vi "Import FPGA Addon Configuration.vi"(8 "error in":errorcluster, 10 "configuration file path":path, 11 "FPGA addon refnum in":T1=18446744073709551615 format="%.0x") -> (0 "error out":errorcluster, 3 "FPGA addon refnum out":T1=18446744073709551615 format="%.0x")   [LabVIEW 2020, in "Scripting API.lvlib"]
doc: "Imports and applies the FPGA addon configuration to the target custom device. The wired path must lead to a valid \".dat\" file, otherwise this VI will return an error."
uses:
  Scripting API.lvlib
  <vilib>/NI VeriStand/Custom Device API/Custom Device Item Ref.ctl
  Addon/Addon Shared/Types/FG Action.ctl
  Addon/Addon Shared/Types/FPGA Settings.ctl
  Addon/Addon Shared/SubVIs/Constants.vi
  <vilib>/NI VeriStand/Custom Device API/NI VeriStand - Get Item Property.vi
  <vilib>/NI VeriStand/Custom Device API/Get Item Property (Path).vi
  <vilib>/NI VeriStand/Custom Device API/Get Item Property (String).vi
  <vilib>/NI VeriStand/Custom Device API/Get Item Property (Boolean).vi
  <vilib>/NI VeriStand/Custom Device API/NI VeriStand - Set Item Property.vi
  <vilib>/NI VeriStand/Custom Device API/Set Item Property (Path).vi
  <vilib>/NI VeriStand/Custom Device API/Set Item Property (String).vi
  <vilib>/NI VeriStand/Custom Device API/Set Item Property (Boolean).vi
  <vilib>/NI/NI VeriStand Custom Device Import and Export Tool/ImportExport.lvlib
  Addon/Addon Shared/FPGA Addon Shared.lvlib
  <vilib>/NI VeriStand/Custom Device API/Custom Device API.lvlib
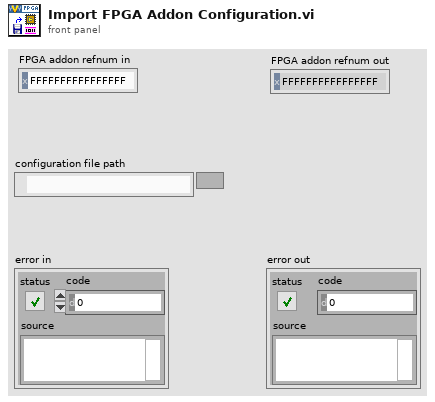
[diagram p1: front panel]
types:
  T1 = typedef "Custom Device API.lvlib/Custom Device Item Ref.ctl" = u64
  T2 = typedef "FPGA Addon Shared.lvlib/FPGA Settings.ctl" = cluster{"Bitfile path":path, "RIO Device Address":string, "Group":bool}
  T3 = typedef "FPGA Addon Shared.lvlib/FG Action.ctl" = enum8{"GET", "SET"}
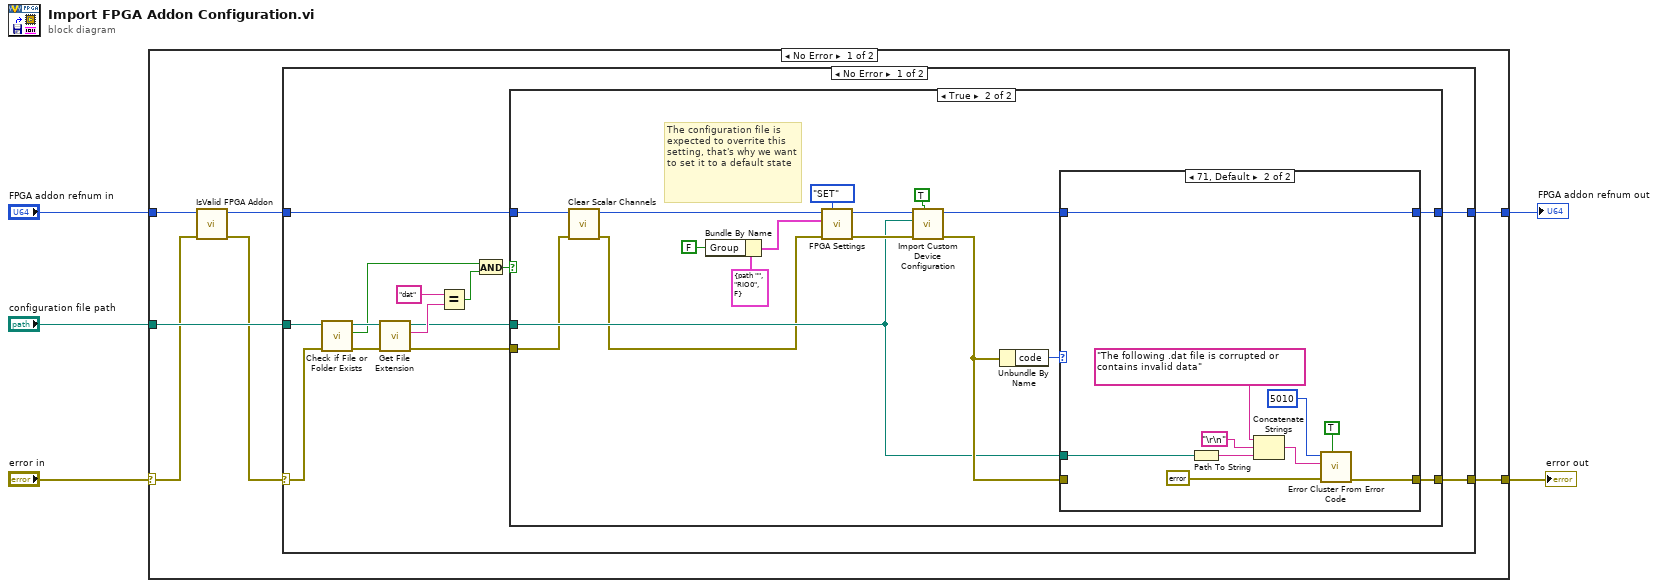
[diagram p0: block diagram]
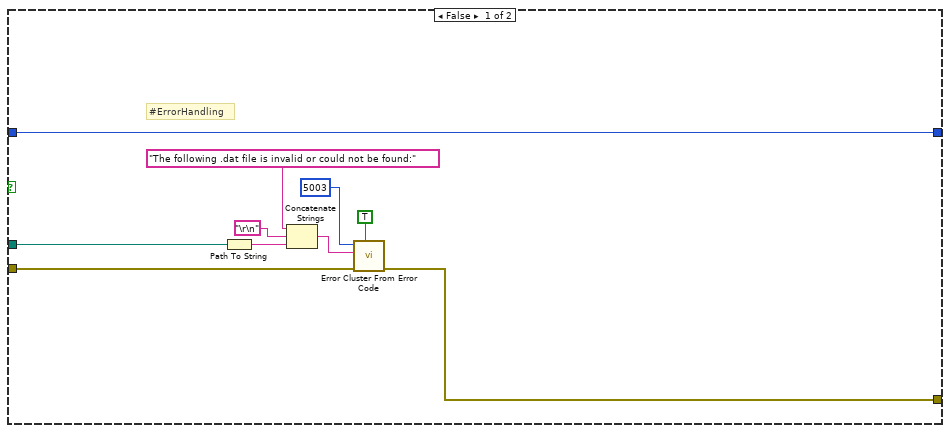
[diagram p2: hidden frame]
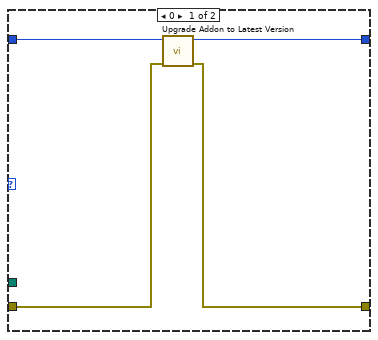
[diagram p3: hidden frame]
diagram:
  n1 = case shown="No Error" "error in" {
    selector: "error in" -> [w10 w70]
    tunnel: "FPGA addon refnum in" -> [w12 w71]
    tunnel: "configuration file path" -> [w11 _]
    tunnel: [w8 w71] -> w2
    tunnel: [w7 w70] -> w1
    frame No Error {
      n2 = call "IsValid FPGA Addon.vi"("error in"=w10, "FPGA Addon refnum in"=w12) -> ("error out"=w6:errorcluster, "FPGA Addon refnum out"=w9:T1)  [unwired: 8 in]
      n3 = case shown="No Error" w6 {
        selector: w6 -> [w15 w69]
        tunnel: w11 -> [w21 _]
        tunnel: w9 -> [w20 w68]
        tunnel: [w18 w68] -> w8
        tunnel: [w17 w69] -> w7
        frame No Error {
          n4 = call <vilib>:"Check if File or Folder Exists.vi"("error in (no error)"=w15, "path"=w21) -> ("error out"=w26:errorcluster, "file or folder exists?"=w24:bool, "dup path"=w25:path)  [unwired: 7 in]
          n5 = call <vilib>:"Get File Extension.vi"("error in (no error)"=w26, "file"=w25) -> ("error out"=w19:errorcluster, "lowercase file extension"=w14:string, "dup file"=w13:path)  [unwired: 5 in, 2 out]
          n6 = Equal?(x="dat", y=w14) -> (x = y?=w22:bool)
          n7 = And(x=w24, y=w22) -> (x .and. y?=w16:bool)
          n8 = case shown="True" w16 {
            tunnel: w20 -> [w31 w42]
            tunnel: w19 -> [w30 w41]
            tunnel: [w31 w37] -> w18
            tunnel: [w29 w44] -> w17
            tunnel: w13 -> [w28 w43]
            frame False {
              # "#ErrorHandling"
              n9 = Path To String(path=w28) -> (string=w35:string)
              n10 = Concatenate Strings("The following .dat file is invalid or could not be found:" ("error message (\"\")"), "\r\n", w35) -> (w36:string)
              n11 = call <vilib>:"Error Cluster From Error Code.vi"("show call chain? (False)"=TRUE, "error in (no error)"=w30, "error message (\"\")"=w36, "error code (0)"=5003) -> ("error out"=w29:errorcluster)  [unwired: 5 in]
            }
            frame True {
              # "The configuration file is expected to overrite this setting, that's why we want to set it to a default state"
              n12 = call "Clear Scalar Channels.vi"("error in"=w41, "FPGA Addon refnum in"=w42) -> ("error out"=w39:errorcluster, "FPGA Addon refnum out"=w40:T1)  [unwired: 8 in]
              n13 = Bundle By Name(cluster=T2 {"Bitfile path"=path "", "RIO Device Address"="RIO0", "Group"=FALSE} ("FPGA Settings"), "Group"=FALSE) -> (w52:T2)
              n14 = call "FPGA Settings.vi"("Action"=FG_Action."SET", "error in (no error)"=w39, "FPGA Settings"=w52, "Item Ref"=w40) -> ("error out"=w47:errorcluster, "Item Ref out"=w48:T1)  [unwired: 5 in, 1 out]
              n15 = call <vilib>:"Import Custom Device Configuration.vi"("Overwrite Existing?"=TRUE, "error in (no error)"=w47, "Path"=w43, "NodeID"=w48) -> ("error out"=w45:errorcluster, "NodeID out"=w38:u64)  [unwired: 5 in, 1 out]
              n16 = Unbundle By Name(w45) -> ("code"=w46:i32)
              n17 = case shown="71, Default" w46 {
                tunnel: w45 -> [w55 _]
                tunnel: [w54 w61] -> w44
                tunnel: w43 -> [_ w60]
                tunnel: w38 -> [w57 w58]
                tunnel: [w56 w58] -> w37
                frame 0 {
                  n18 = call "Upgrade Addon to Latest Version.vi"("error in (no error)"=w55, "Device Item Ref in in"=w57) -> ("error out"=w54:errorcluster, "Device Item Ref out"=w56:T1)  [unwired: 8 in]
                }
                frame 71, Default {
                  n19 = Path To String(path=w60) -> (string=w66:string)
                  n20 = Concatenate Strings("The following .dat file is corrupted or contains invalid data" ("error message (\"\")"), "\r\n", w66) -> (w67:string)
                  n21 = call <vilib>:"Error Cluster From Error Code.vi"("show call chain? (False)"=TRUE, "error in (no error)"=errorcluster {"status"=FALSE, "code"=0, "source"=""}, "error message (\"\")"=w67, "error code (0)"=5010) -> ("error out"=w61:errorcluster)  [unwired: 5 in]
                }
              }
            }
          }
        }
        frame Error {
        }
      }
    }
    frame Error {
    }
  }
  "error out" <- w1
  "FPGA addon refnum out" <- w2
